vi "Get Bitfile Scalars.vi"(8 "error in":errorcluster, 11 "FPGA addon refnum in":T3=18446744073709551615 format="%.0x") -> (0 "error out":errorcluster, 2 "bitfile scalars out":T1[](array[typedef]), 3 "FPGA addon refnum out":T3=18446744073709551615 format="%.0x")   [LabVIEW 2020, in "Scripting API.lvlib"]
doc: "Returns a data array containing information about the available control and indicator registers within the bitfile. The function checks as well wether a given control or indicator was already imported (and exists as a channel) within the target FPGA addon custom device."
uses:
  Scripting API.lvlib
  <vilib>/NI VeriStand/Custom Device API/Custom Device Item Ref.ctl
  TypeDefs/Output Scalar Data.ctl
  Addon/Addon Shared/Types/FPGA Addon Data Type.ctl
  Addon/Addon Shared/SubVIs/Constants.vi
  <vilib>/NI/NI VeriStand Advanced SysDef API/_SubVIs/SysDef.Search.GUID.vi
  Addon/Addon Shared/FPGA Addon Shared.lvlib
  <vilib>/NI/NI VeriStand Advanced SysDef API/SysDef API/Advanced System Definition.lvlib
  <vilib>/NI VeriStand/Custom Device API/Custom Device API.lvlib
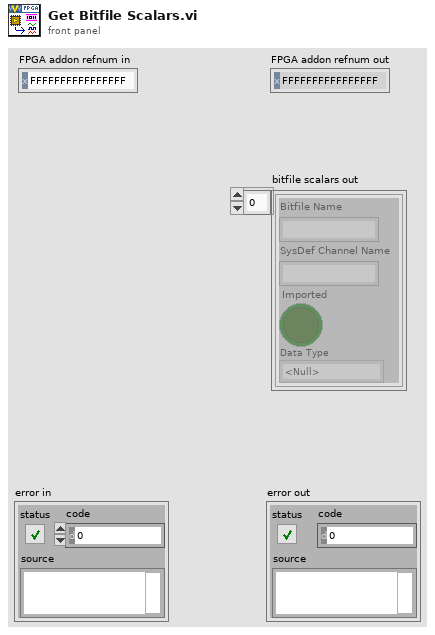
[diagram p1: front panel]
types:
  T1 = typedef "Scripting API.lvlib/Output Scalar Data.ctl" = cluster{"Bitfile Name":string, "SysDef Channel Name":string, "Imported":bool, "Data Type":T2}
  T2 = typedef "FPGA Addon Shared.lvlib/FPGA Addon Data Type.ctl" = enum8{"<Null>", "I8", "I16", "I32", "I64", "U8", "U16", "U32", "U64", "SGL", "Boolean", "Analog PWM In Settings", "Analog PWM In", "Digital PWM In Settings", "Digital PWM In", "Digital PWM Out", "Sine Out", "FXP", "FXP+/-24.5", "FXP+/-16.5", "FXP+/-32.8", "FXP+/-64.32", "FXP+/-16.7", "FXP+/-20.5", "FXP+/-27.5", "FXP+/-32.16", "FXP+16.3", "FXP+18.3", "Digital Static In", "Digital Static Out", "Digital Static In Settings", "Digital WSS Out", "Quad Encoder Settings", "Quad Encoder In", "Group"}
  T3 = typedef "Custom Device API.lvlib/Custom Device Item Ref.ctl" = u64
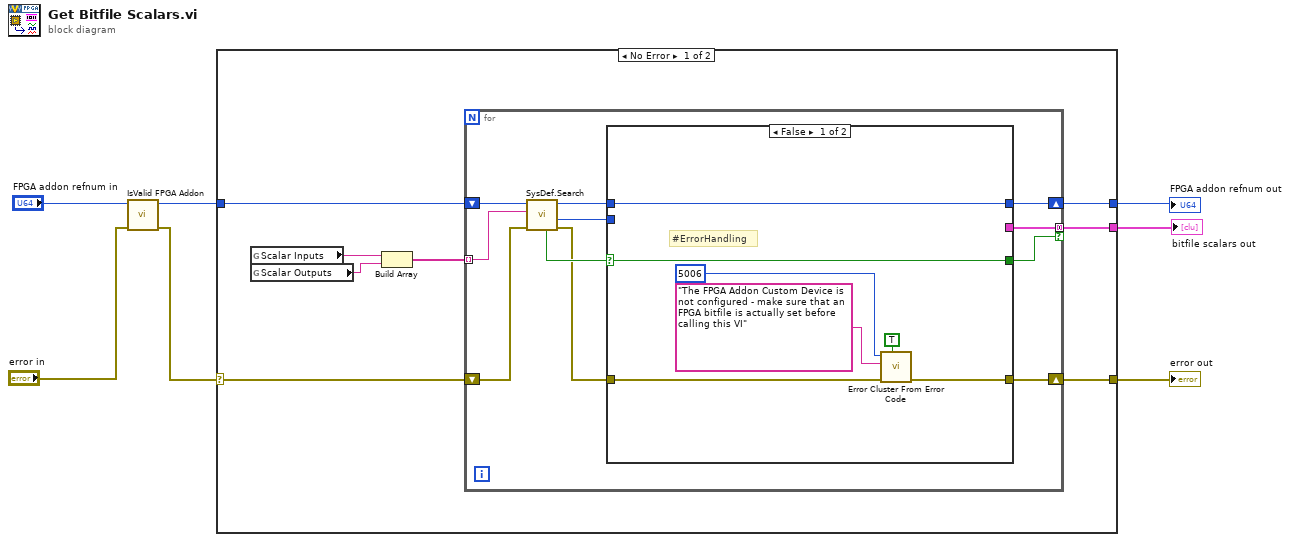
[diagram p0: block diagram]
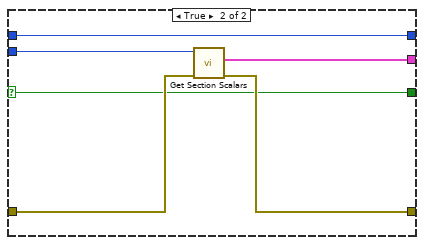
[diagram p2: hidden frame]
diagram:
  n1 = call "IsValid FPGA Addon.vi"("error in"="error in", "FPGA Addon refnum in"="FPGA addon refnum in") -> ("error out"=w4:errorcluster, "FPGA Addon refnum out"=w6:T3)  [unwired: 8 in]
  n2 = case shown="No Error" w4 {
    selector: w4 -> [w11 w40]
    tunnel: w6 -> [w12 w41]
    tunnel: [w10 w41] -> w3
    tunnel: [w9 w40] -> w2
    tunnel: [w8 _] -> w1
    frame No Error {
      n3 = global read "Constants.vi" "Scalar Inputs"() -> (w15:string)
      n4 = global read "Constants.vi" "Scalar Outputs"() -> (w14:string)
      n5 = Build Array(w15, w14) -> (w13:string[])
      n6 = for {
        tunnel: w13 -> [w25] mode=indexing
        shift-right: [w18] -> w9
        shift-left: w11 -> [w21]
        shift-right: [w19] -> w10
        shift-left: w12 -> [w26]
        tunnel: [w17] -> w8 mode=concatenating if=w16
        n7 = call-poly <vilib>:"SysDef.Search.vi"("error in (no error)"=w21, "GUID"=w25, "nodeID"=w26) -> ("error out"=w20:errorcluster, "Value out"=w23:u64, "nodeID out"=w22:u64, "Found?"=w24:bool)  [unwired: 5 in]
        n8 = case shown="False" w24 {
          selector: w24 -> [w32 w34]
          tunnel: w23 -> [_ w39]
          tunnel: w22 -> [w33 w37]
          tunnel: w20 -> [w28 w38]
          tunnel: [w33 w37] -> w19
          tunnel: [w27 w36] -> w18
          tunnel: [_ w35] -> w17
          tunnel: [w32 w34] -> w16
          frame False {
            # "#ErrorHandling"
            n9 = call <vilib>:"Error Cluster From Error Code.vi"("show call chain? (False)"=TRUE, "error in (no error)"=w28, "error message (\"\")"="The FPGA Addon Custom Device is not configured - make sure that an FPGA bitfile is actually set before calling this VI" ("error message (\"\")"), "error code (0)"=5006) -> ("error out"=w27:errorcluster)  [unwired: 5 in]
          }
          frame True {
            n10 = call "Get Section Scalars.vi"("error in"=w38, "section ref in"=w39) -> ("error out"=w36:errorcluster, "section scalars out"=w35:T1[])  [unwired: 7 in, 1 out]
          }
        }
      }
    }
    frame Error {
    }
  }
  "error out" <- w2
  "FPGA addon refnum out" <- w3
  "bitfile scalars out" <- w1
